vi "Get Tx Acyclic Message Configuration.vi"(8 "error in":errorcluster, 10 "configuration string":string, 11 "port":T1 format="%.0x") -> (0 "error out":errorcluster, 2 "configuration string out":string, 3 "port out":T1 format="%.0x")   [LabVIEW 2020, in "Ballard ARINC 429 Hardware Configuration.lvlib"]
uses:
  Ballard ARINC 429 Hardware Configuration.lvlib
  <vilib>/NI VeriStand/Custom Device API/Custom Device Item Ref.ctl
  Constants.vi
  Scripting/Ballard/Ballard ARINC 429 Scripting.lvlib
  Scripting/ARINC 429/ARINC 429 Scripting.lvlib
  <vilib>/NI VeriStand/Custom Device API/Custom Device API.lvlib
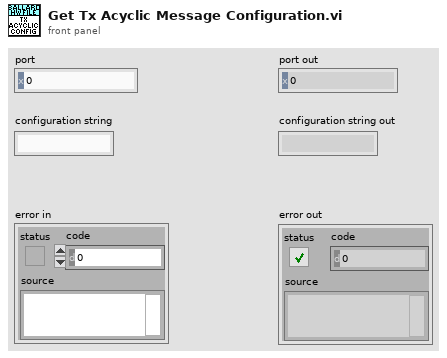
[diagram p1: front panel]
types:
  T1 = typedef "Custom Device API.lvlib/Custom Device Item Ref.ctl" = u64
  T2 = typedef "Label Properties.ctl" = cluster{"label (Dec)":T3, "SDI value":u8, "SDI enabled":bool}
  T3 = typedef "Label.ctl" = u8
  T4 = typedef "Transfer Type.ctl" = enum16{"Scheduled", "Acyclic", "Block", "Strobe"}
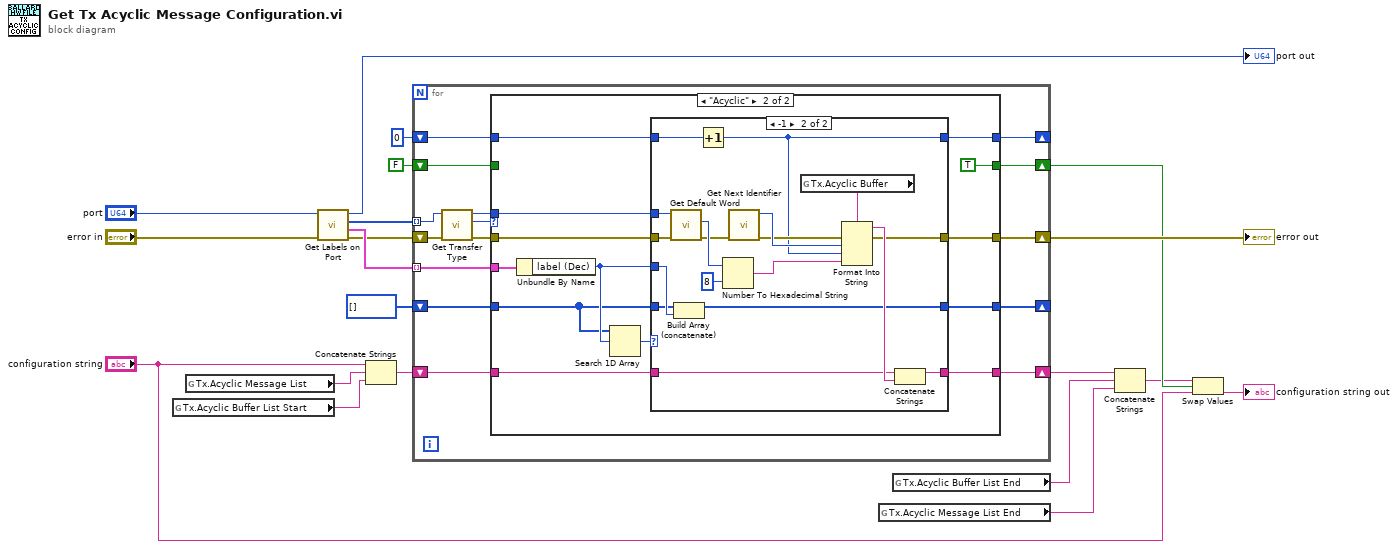
[diagram p0: block diagram]
diagram:
  n1 = global read "Constants.vi" "Tx.Acyclic Buffer List Start"() -> (w5:string)
  n2 = global read "Constants.vi" "Tx.Acyclic Message List"() -> (w6:string)
  n3 = call "Get Labels on Port.vi"("error in"="error in", "port in"="port") -> ("error out"=w14:errorcluster, "labels properties"=w16:T2[], "labels"=w15:T1[], "port out"=→"port out":T1)  [unwired: 6 in]
  n4 = Concatenate Strings("configuration string", w6, w5) -> (w17:string)
  n5 = for {
    shift-right: [w33] -> w10
    shift-left: w17 -> [w34]
    tunnel: w16 -> [w35] mode=indexing
    tunnel: w15 -> [w29] mode=indexing
    shift-right: [w32] -> w13
    shift-left: w14 -> [w31]
    shift-right: [w25] -> w11
    shift-left: FALSE -> [w26]
    shift-right: [w23] -> _
    shift-left: u8[] [] -> [w24]
    shift-right: [w21] -> _
    shift-left: 0 -> [w22]
    n6 = call "Get Transfer Type.vi"("error in"=w31, "label ref in"=w29) -> ("error out"=w30:errorcluster, "transfer type"=w27:T4, "label ref out"=w28:T1)  [unwired: 7 in]
    n7 = case shown="\"Acyclic\"" w27 {
      tunnel: w35 -> [_ w51]
      tunnel: w34 -> [w39 w53]
      tunnel: [w39 w52] -> w33
      tunnel: [w40 w47] -> w32
      tunnel: w30 -> [w40 w49]
      tunnel: w28 -> [_ w48]
      tunnel: w26 -> [w38 _]
      tunnel: [w38 TRUE] -> w25
      tunnel: w24 -> [w37 w43]
      tunnel: [w37 w44] -> w23
      tunnel: w22 -> [w36 w42]
      tunnel: [w36 w41] -> w21
      frame Default {
      }
      frame "Acyclic" {
        n8 = Unbundle By Name(w51) -> ("label (Dec)"=w46:T3)
        n9 = Search 1D Array(1D array=w43, element=w46) -> (index of element=w45:i32)  [unwired: 1 in]
        n10 = case shown="-1" w45 {
          tunnel: w53 -> [w56 w71]
          tunnel: [w56 w70] -> w52
          tunnel: w49 -> [w57 w68]
          tunnel: w48 -> [_ w67]
          tunnel: [w57 w61] -> w47
          tunnel: w46 -> [_ w65]
          tunnel: [w55 w64] -> w44
          tunnel: w43 -> [w55 w63]
          tunnel: w42 -> [w54 w59]
          tunnel: [w54 w58] -> w41
          frame Default {
          }
          frame -1 {
            n11 = call "Get Default Word.vi"("error in"=w68, "Item Ref in"=w67) -> ("error out"=w66:errorcluster, "default word"=w74:u32)  [unwired: 7 in, 1 out]
            n12 = Build Array (concatenate)(w63, w65) -> (w64:T3[])
            n13 = Increment(x=w59) -> (x+1=w58:i32)
            n14 = Number To Hexadecimal String(1:i16 8 ("width (-)"), 2:w74) -> (0:w69:string)
            n15 = call "Get Next Identifier.vi"("error in"=w66) -> ("error out"=w62:errorcluster, "ID"=w75:u32)  [unwired: 9 in]
            n16 = global read "Constants.vi" "Tx.Acyclic Buffer"() -> (w60:string)
            n17 = Format Into String(format string=w60, error in=w62, w75, w58, w69) -> (resulting string=w72:string, error out=w61:errorcluster)  [unwired: 1 in]
            n18 = Concatenate Strings(w71, w72) -> (w70:string)
          }
        }
      }
    }
  }
  "error out" <- w13
  n19 = global read "Constants.vi" "Tx.Acyclic Message List End"() -> (w4:string)
  n20 = global read "Constants.vi" "Tx.Acyclic Buffer List End"() -> (w3:string)
  n21 = Concatenate Strings(w10, w3, w4) -> (w9:string)
  n22 = Swap Values(12:w9, 13:w11, 14:"configuration string") -> (3:→"configuration string out":string)  [unwired: 1 out]
